vi "Virtual DAQ Signal erfassen.vi"(0 "Messart":T1(ring), 1 "Physikalischer Kanal":string, 2 "PFI Klemme":string, 3 "Abtastrate Hz":dbl=1000.0, 4 "Samples pro Block":i32=100, 5 "Spannungsbereich ±V":dbl=10.0, 6 "Kontinuierlich":bool, 7 "Ausgabewerte":dbl[](array[numeric])) -> (20 "Signal":waveform(dbl)(graph), 21 "Daten":dbl[](array[numeric]), 22 "Status":dbl, 27 "error out":errorcluster)   [LabVIEW 2026]
doc: "Bedien-VI fuer die Steckwerkbank. Messart, physikalischen Kanal und Timing waehlen. Ausgabewerte sind einzelne Portwerte oder ein analoger Datenblock. Bedien-VI einmal ausfuehren oder PuT3 DAQ.vi in eigener Schleife aufrufen."
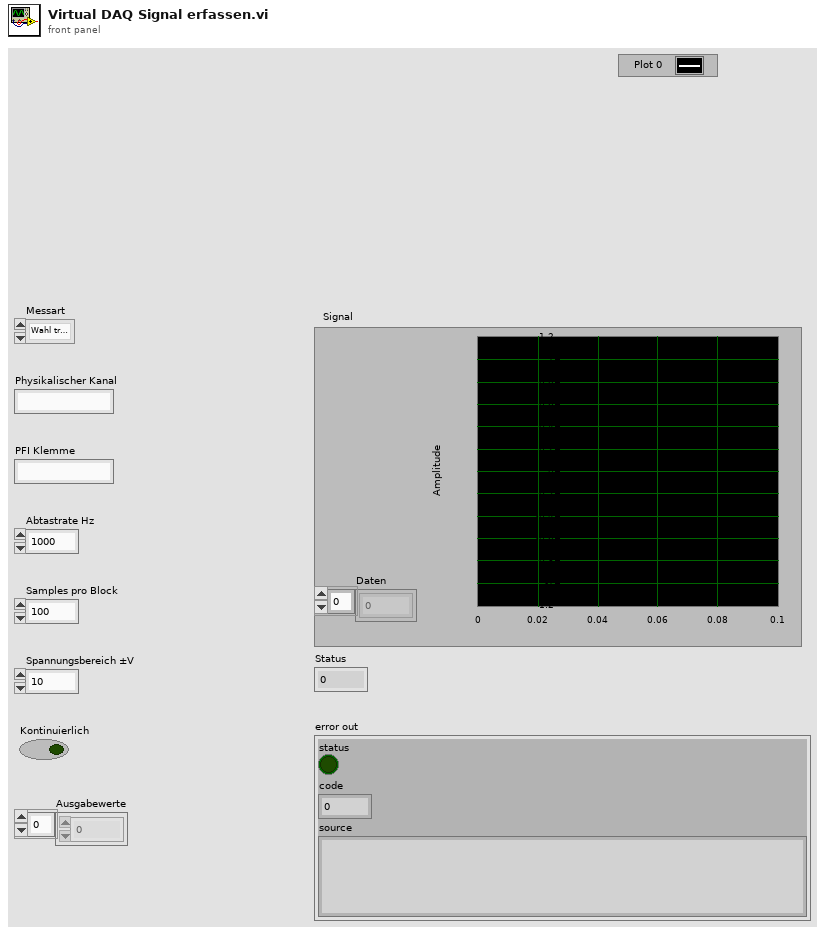
[diagram p1: front panel]
types:
  T1 = enum8{"Wahl treffen", "AI Spannung", "AO Spannung", "DI Lesen", "DO Schreiben", "CTR Frequenz", "DMM Widerstand", "Ausgaenge freigeben"}
  T2 = cluster{"Messart":enum8{"Wahl treffen", "AI Spannung", "AO Spannung", "DI Lesen", "DO Schreiben", "CTR Frequenz", "DMM Widerstand", "Ausgaenge freigeben"}, "Kanal":string, "PFI":string, "Rate":dbl, "Samples":i32, "Bereich":dbl, "Kontinuierlich":bool}
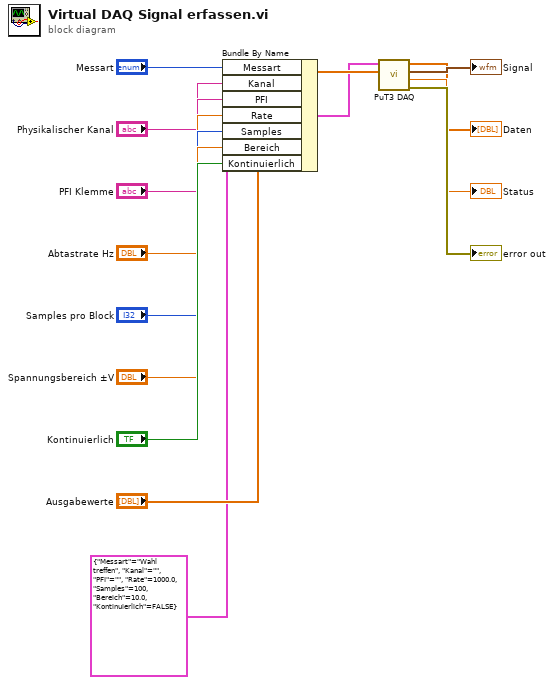
[diagram p0: block diagram]
diagram:
  n1 = Bundle By Name(cluster=T2 {"Messart"=enum."Wahl treffen", "Kanal"="", "PFI"="", "Rate"=1000.0, "Samples"=100, "Bereich"=10.0, "Kontinuierlich"=FALSE}, "Messart"="Messart", "Kanal"="Physikalischer Kanal", "PFI"="PFI Klemme", "Rate"="Abtastrate Hz", "Samples"="Samples pro Block", "Bereich"="Spannungsbereich ±V", "Kontinuierlich"="Kontinuierlich") -> (w9:T2)
  n2 = call "PuT3 DAQ.vi"("Ausgabewerte"="Ausgabewerte", "Auftrag"=w9) -> ("error out"=→"error out":errorcluster, "Status"=→"Status":dbl, "Signal"=→"Signal":waveform(dbl), "Daten"=→"Daten":dbl[])  [unwired: 6 in]
